vi "Generate Plots.vi"(6 "Y Errors":dbl[](array[numeric]), 7 "X Errors":dbl[](array[numeric]), 9 "Y Data":dbl[](array[numeric]), 11 "X Data":dbl[](array[numeric])) -> (3 "Plot Data":cluster{"X Data":dbl[], "Y Data":dbl[]}[](array[cluster]))   [LabVIEW 2012, in "XY Plot with Error Bars.xctl"]
uses:
  XY Plot with Error Bars.xctl
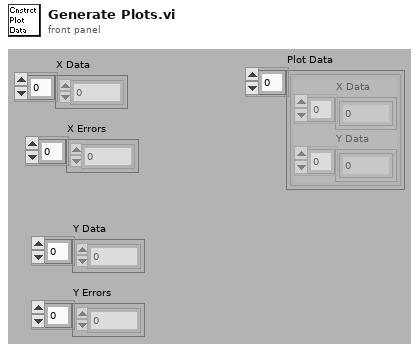
[diagram p1: front panel]
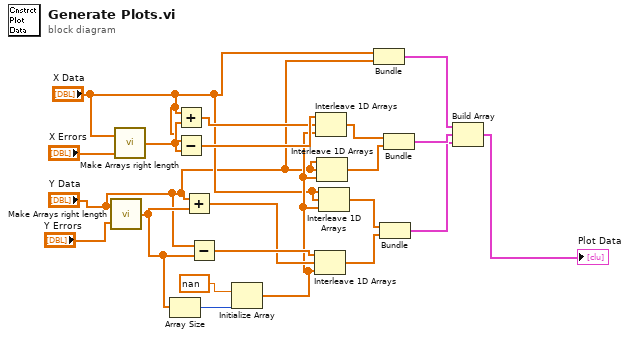
[diagram p0: block diagram]
diagram:
  n1 = call "Make Arrays right length.vi"("Errors"="Y Errors", "Data"="Y Data") -> ("Errors[1..len(Data)]"=w19:dbl[])
  n2 = call "Make Arrays right length.vi"("Errors"="X Errors", "Data"="X Data") -> ("Errors[1..len(Data)]"=w14:dbl[])
  n3 = Array Size(array=w19) -> (size(s)=w18:i32)
  n4 = Add(x="X Data", y=w14) -> (x+y=w12:dbl[])
  n5 = Subtract(x="X Data", y=w14) -> (x-y=w13:dbl[])
  n6 = Add(x="Y Data", y=w19) -> (x+y=w15:dbl[])
  n7 = Subtract(x="Y Data", y=w19) -> (x-y=w16:dbl[])
  n8 = Initialize Array(nan, w18) -> (w11:dbl[])
  n9 = Interleave 1D Arrays(w16, w15, w11) -> (w5:dbl[])
  n10 = Interleave 1D Arrays(w13, w12, w11) -> (w8:dbl[])
  n11 = Interleave 1D Arrays("Y Data", "Y Data", w11) -> (w7:dbl[])
  n12 = Interleave 1D Arrays("X Data", "X Data", w11) -> (w6:dbl[])
  n13 = Bundle("X Data"="X Data", "Y Data"="Y Data") -> (w4:cluster{"X Data":dbl[], "Y Data":dbl[]})  [unwired: 1 out]
  n14 = Bundle(w6, w5) -> (w2:cluster{dbl[], dbl[]})  [unwired: 1 out]
  n15 = Bundle(w8, w7) -> (w3:cluster{dbl[], dbl[]})  [unwired: 1 out]
  n16 = Build Array(w4, w3, w2) -> (→"Plot Data":cluster{"X Data":dbl[], "Y Data":dbl[]}[])
